vi "uService List Init.vi"(8 "error in (no error)":errorcluster, 11 "Guardian in":refnum<class "Guardian.lvclass">) -> (0 "error out":errorcluster, 3 "Guardian out":refnum<class "Guardian.lvclass">)   [LabVIEW 2020, in "TALOS.lvlib" / "Guardian.lvlib" / "Guardian.lvclass"]
uses:
  Guardian.lvclass
  Guardian.lvclass/Guardian.ctl
  Classes/uService List/uService List.lvclass
  Classes/Distributed uService Map/Distributed uService Map.lvclass
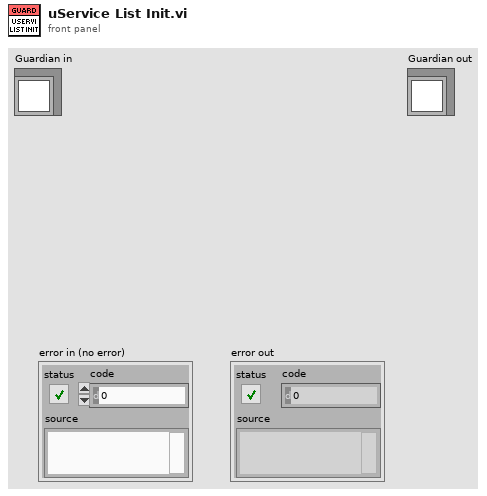
[diagram p1: front panel]
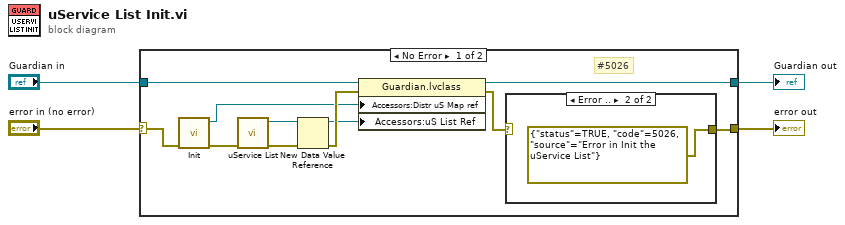
[diagram p0: block diagram]
diagram:
  n1 = case shown="No Error" "error in (no error)" {
    selector: "error in (no error)" -> [w11 w18]
    tunnel: [w8 w18] -> w4
    tunnel: "Guardian in" -> [w7 w19]
    tunnel: [w13 w19] -> w1
    frame No Error {
      # "#5026"
      n2 = call "Init.vi"("error in (no error)"=w11) -> ("error out"=w10:errorcluster, "Distr uS Map ref out"=w5:refnum<data-value>)  [unwired: 9 in]
      n3 = call-poly "uService List.vi"("error in (no error)"=w10) -> ("error out"=w14:errorcluster, "uService out"=w15:refnum<class "uService List.lvclass">)  [unwired: 9 in]
      n4 = New Data Value Reference(data value=w15, error in=w14) -> (data value reference=w6:refnum<data-value>, error out=w12:errorcluster)
      n5 = property class="Guardian.lvclass"(reference=w7, error in=w12, "Accessors:Distr uS Map ref"=w5, "Accessors:uS List Ref"=w6) -> (reference out=w13:refnum<class "Guardian.lvclass">, error out=w9:errorcluster)
      n6 = case shown="Error .." w9 {
        selector: w9 -> [w16 _]
        tunnel: [w16 errorcluster {"status"=TRUE, "code"=5026, "source"="Error in Init the uService List"} ("error IO")] -> w8
        frame No Error {
        }
        frame Error {
        }
      }
    }
    frame Error {
    }
  }
  "error out" <- w4
  "Guardian out" <- w1
